vi "Convert mystery V to mystery output.vi"(11 "Waveform":dbl) -> (3 "Numeric":dbl)   [LabVIEW 2024]
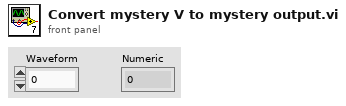
[diagram p1: front panel]
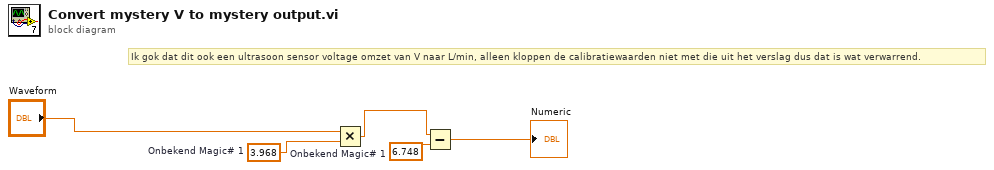
[diagram p0: block diagram]
diagram:
  w4 = 6.748  # Onbekend Magic# 1
  w3 = 3.968  # Onbekend Magic# 1
  # "Ik gok dat dit ook een ultrasoon sensor voltage omzet van V naar L/min, alleen kloppen de calibratiewaarden niet met die uit het verslag dus dat is wat verwarrend."
  n1 = Multiply(x="Waveform", y=w3) -> (x*y=w2:dbl)
  n2 = Subtract(x=w2, y=w4) -> (x-y=→"Numeric":dbl)
